vi "Battery_Test_System_Simulation.vi"() -> ()   [LabVIEW 2019]
uses:
  <vilib>/numeric/Random Number (Range) U64.vi
  <vilib>/numeric/sub_Random U32.vi
panel:
  out "Clock":string
  in  "Save Button":bool
  out "Cycle":dbl(slide)=1.0 scale=0.0..10.0
  in  "Stop Button":bool
  in  "Close Button":bool
  out "Temperature":dbl
  out "Temperature":dbl[](graph)
  out "DC Current":dbl
  out "DC Voltage":dbl
  out "DC Current":u64(graph) caption="Waveform Chart - Dark"
  out "DC Voltage":u64(graph) caption="Waveform Chart - Dark"
  in  "Start Button":bool
  in  "Tab Control":enum32{"Charge", "Discharge"}(tab)
  in  "Charge Duration":dbl
  in  "Charge Current":dbl
  in  "C-Rate":dbl
  in  "Charging Voltage":dbl
  in  "Charge Duration 2":dbl
  in  "Charge Current 2":dbl
  in  "C-Rate 2":dbl
  in  "DisCharging Voltage 2":dbl
  in  "Select Function":enum32{"Button 1", "Button 2"}(radio)
  out "DC Load Connected?":bool
  out "Power Supply Connected?":bool
  out "DAQ CONNECTED?":bool
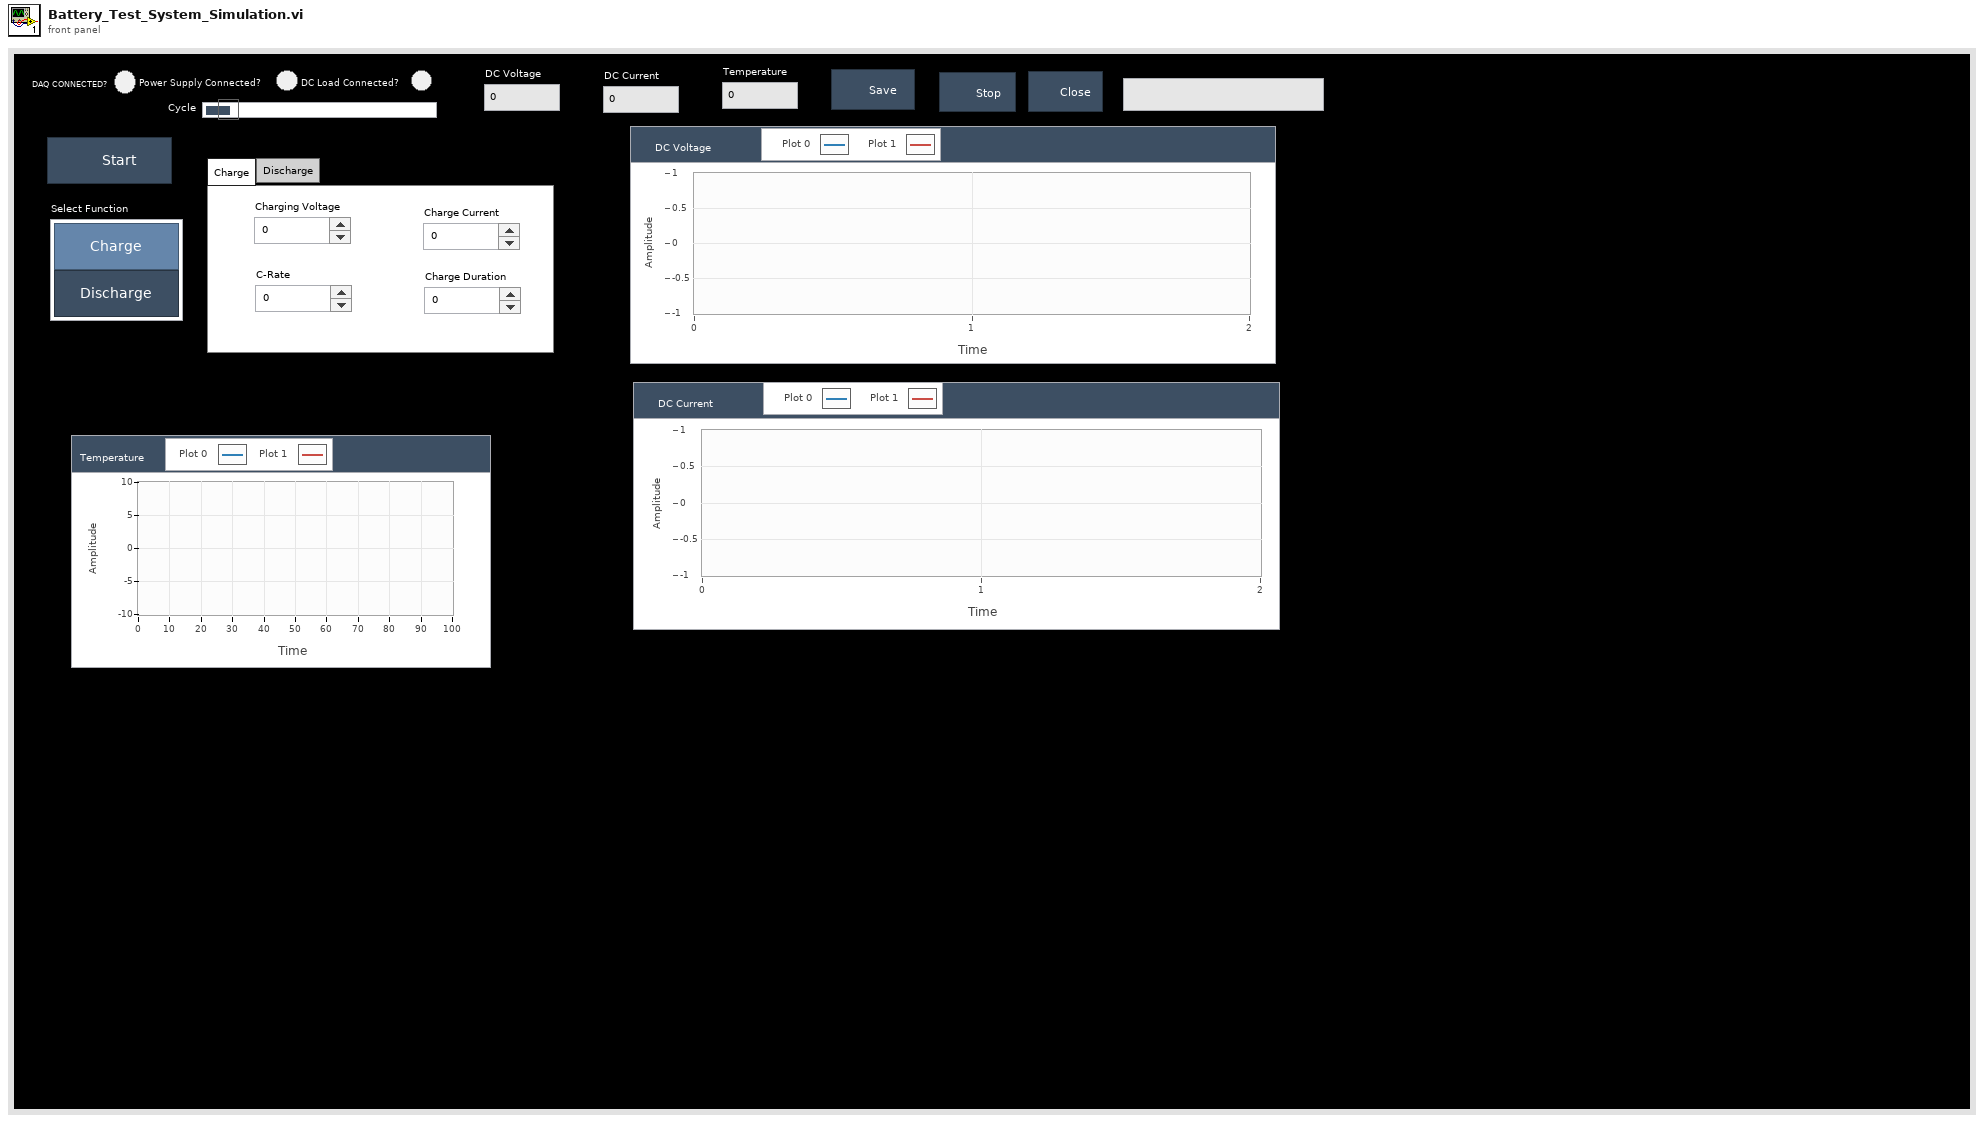
[diagram p1: front panel]
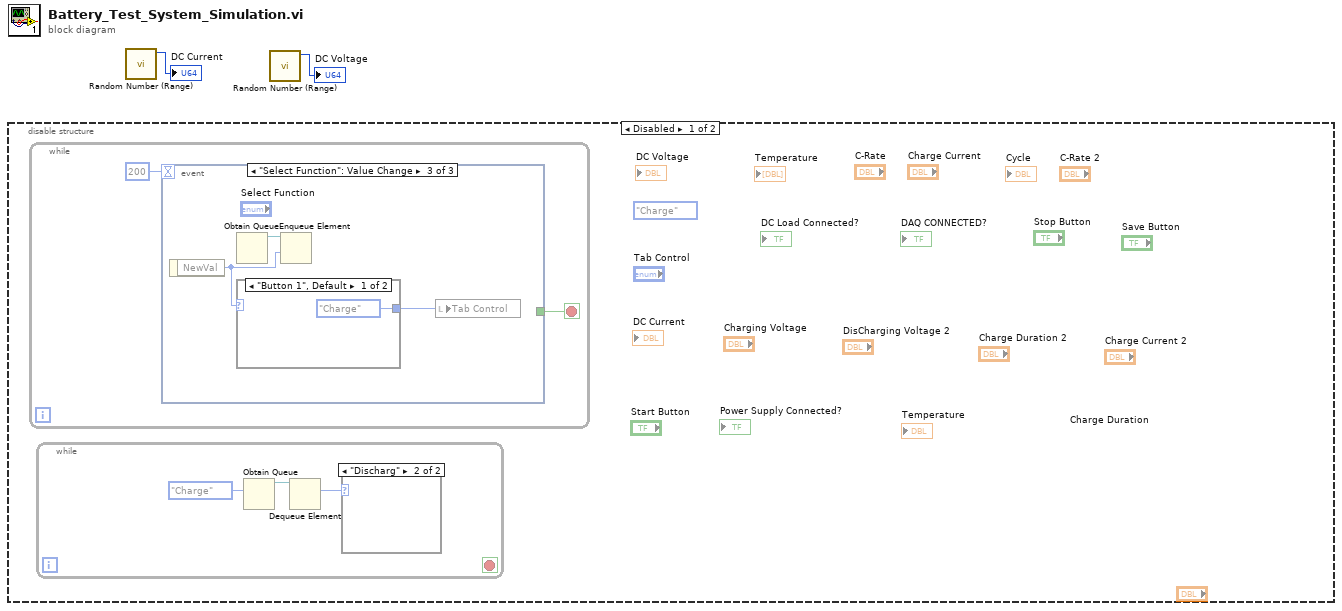
[diagram p0: block diagram]
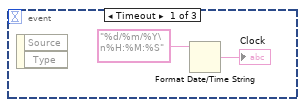
[diagram p2: hidden frame]
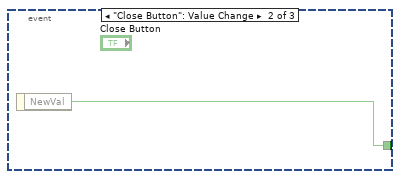
[diagram p3: hidden frame]
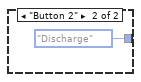
[diagram p4: hidden frame]
diagram:
  n1 = disable-structure shown="Disabled" {
    frame Disabled {
      (unwired) enum16{"Charge", "Discharge"}."Charge" ("Enum")
      n2 = while {
        stop <- w3 stop-if-true
        n3 = event shown="[2] \"Select Function\": Value Change" {
          selector: _ -> [_ _ _]
          dyn-events: _ -> [_ _ _]
          timeout: 200 -> [_ _ _]
          tunnel: [_ w7 _] -> w3
          event Timeout {
            n4 = event-data() -> ()  [unwired: 1 in, 2 out]
            n5 = Format Date/Time String(time format string (%c)="%d/%m/%Y\n%H:%M:%S") -> (date/time string=→"Clock":string)  [unwired: 2 in]
          }
          event "Close Button": Value Change {
            n6 = event-data() -> ("NewVal"=w7:bool)  [unwired: 1 in]
          }
          event "Select Function": Value Change {
            n7 = event-data() -> ("NewVal"=w8:enum32{"Button 1", "Button 2"})  [unwired: 1 in]
            n8 = Obtain Queue() -> (queue out=w9:refnum<queue>)  [unwired: 5 in, 2 out]
            n9 = case shown="\"Button 1\", Default" w8 {
              tunnel: [enum32{"Charge", "Discharge"}."Charge" ("Tab Control") enum32{"Charge", "Discharge"}."Discharge" ("Tab Control")] -> w10
              frame "Button 1", Default {
              }
              frame "Button 2" {
              }
            }
            n10 = Enqueue Element(queue=w9, timeout in ms (-1)=w8) -> ()  [unwired: 2 in, 3 out]
            n11 = local write "Tab Control"(w10) -> ()
          }
        }
      }
      n12 = while {
        stop <- _ stop-if-true
        n13 = Obtain Queue(element data type=enum16{"Charge", "Discharg"}."Charge") -> (queue out=w14:refnum<queue>)  [unwired: 4 in, 2 out]
        n14 = Dequeue Element(queue=w14) -> (element=w13:enum16{"Charge", "Discharg"})  [unwired: 2 in, 3 out]
        n15 = case shown="\"True\"" w13 {
          frame "Charge", Default {
          }
          frame "Discharg" {
          }
        }
      }
    }
    frame Enabled {
    }
  }
  n16 = call-poly <vilib>:"Random Number (Range).vi"() -> ("number"=→"DC Current":u64)  [unwired: 11 in]
  n17 = call-poly <vilib>:"Random Number (Range).vi"() -> ("number"=→"DC Voltage":u64)  [unwired: 11 in]
